vi "mainOCR.vi"() -> ()   [LabVIEW 2025]
uses:
  ocr/ocrParameters.ctl
  ocr/ocr.lvclass
  D:/Test/adslvPackageDev/adstoolkit/tcv/tcv.lvclass
panel:
  out "loadImgSucc":string
  out "succ 2":i32
  in  "Default Parameters":bool
  in  "device":enum16{"CPU", "GPU0"}(ring)
  out "InitRecDec Success":string
  out "SetDevice":string
  in  "ocrParameters":T1={"targetSize"=1088, "expandRatio "=1.12, "padPixels "=10, "binThresh"=0.3, "txt_score_thresh"=0.25, "minArea"=12, "cropMargin"=5, "binSize"=32}
  in  "PathImage":path=path "D:/Test/dllTest/images_2"
  out "Image":T2(plugin-control)
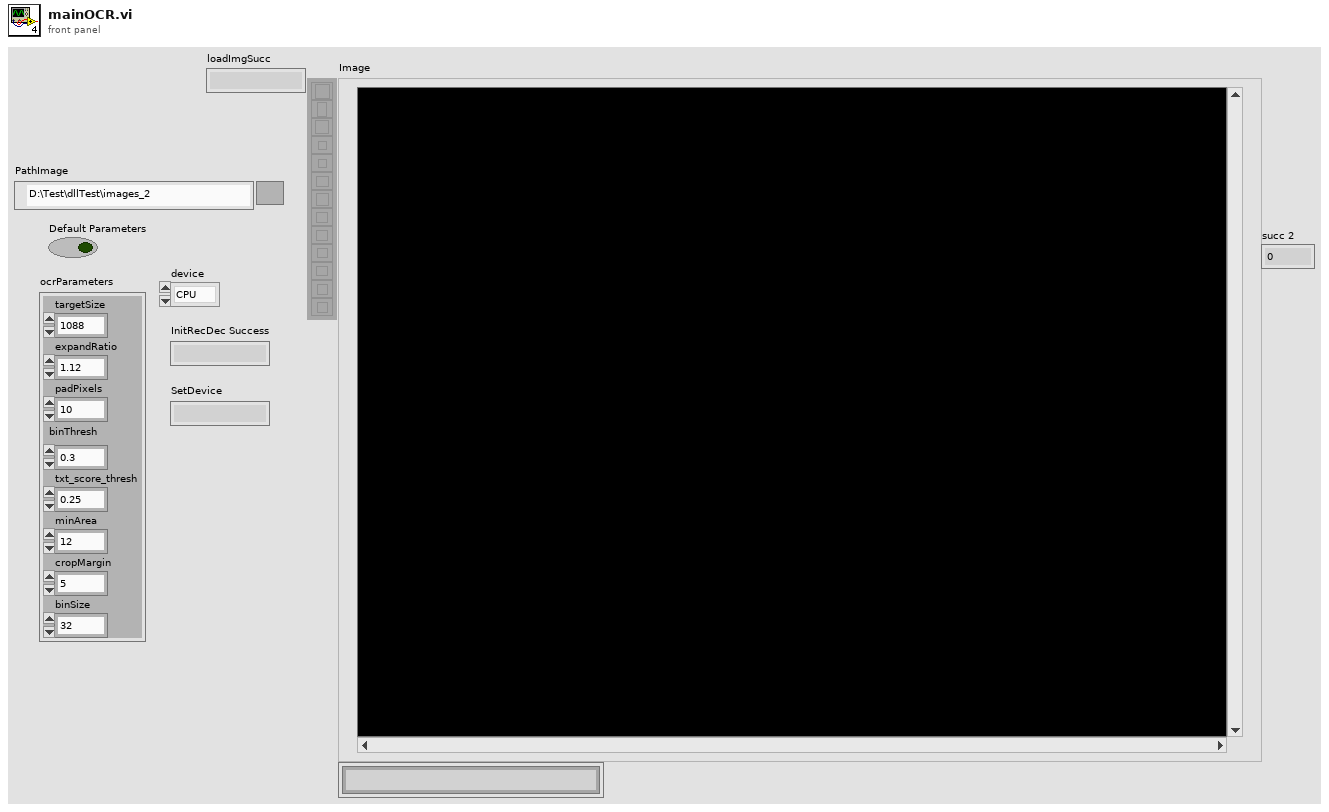
[diagram p1: front panel]
types:
  T1 = typedef "adsOCR.lvlib/ocr.lvclass/ocrParameters.ctl" = cluster{"targetSize":i32, "expandRatio ":sgl, "padPixels ":i32, "binThresh":sgl, "txt_score_thresh":sgl, "minArea":i32, "cropMargin":i32, "binSize":i32}
  T2 = typedef "IMAQ Image.ctl" = refnum<image>
  T3 = typedef "adsOCR.lvlib/ocr.lvclass/TextDecRecResult2L.ctl" = cluster{"imgIdx":i32, "TLx":i32, "TLy":i32, "BRx":i32, "BRy":i32, "angle":sgl, "txtLen":i32}
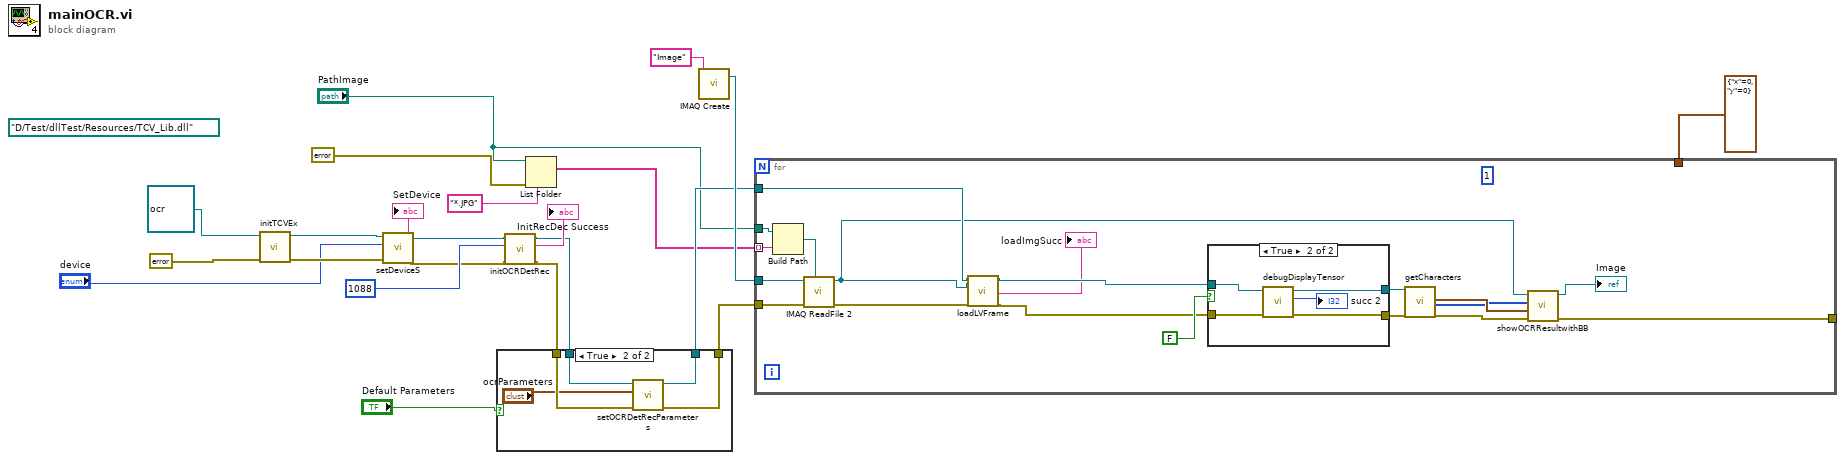
[diagram p0: block diagram]
diagram:
  (unwired) path "D:/Test/dllTest/Resources/TCV_Lib.dll" ("path in")
  n1 = call-dynamic "initTCVEx.vi"("error in (no error)"=errorcluster {"status"=FALSE, "code"=0, "source"=""}, "tcv in"=refnum<class "ocr.lvclass"> refnum ("ocr in")) -> ("error out"=w15:errorcluster, "tcv out"=w16:refnum<class "ocr.lvclass">)  [unwired: 8 in]
  n2 = call-dynamic "setDeviceS.vi"("error in (no error)"=w15, "devices"="device", "tcv in"=w16) -> ("error out"=w4:errorcluster, "SetDevice"=→"SetDevice":string, "tcv out"=w5:refnum<class "ocr.lvclass">)  [unwired: 6 in]
  n3 = call "initOCRDetRec.vi"("error in (no error)"=w4, "targetSize"=1088, "tcv in"=w5) -> ("error out"=w2:errorcluster, "InitRecDec Success"=→"InitRecDec Success":string, "ocr out"=w1:refnum<class "ocr.lvclass">)  [unwired: 5 in, 1 out]
  n4 = case shown="True" "Default Parameters" {
    tunnel: w1 -> [w24 w29]
    tunnel: [w24 w28] -> w14
    tunnel: w2 -> [w23 w27]
    tunnel: [w23 w26] -> w13
    frame False {
    }
    frame True {
      n5 = call-dynamic "setOCRDetRecParameters.vi"("error in (no error)"=w27, "ocrParameters"="ocrParameters", "ocr in"=w29) -> ("error out"=w26:errorcluster, "ocr out"=w28:refnum<class "ocr.lvclass">)  [unwired: 5 in, 2 out]
    }
  }
  n6 = List Folder(path="PathImage", pattern="*.JPG", error in=errorcluster {"status"=FALSE, "code"=0, "source"=""}) -> (filenames=w9:string[])  [unwired: 1 in, 3 out]
  n7 = call "IMAQ Create"("Image Name"="Image") -> ("New Image"=w21:T2)  [unwired: 4 in, 1 out]
  n8 = for {
    tunnel: "PathImage" -> [w48]
    tunnel: w21 -> [w46]
    tunnel: cluster{"x":i32, "y":i32} {"x"=0, "y"=0} -> [_]
    tunnel: w14 -> [w37]
    tunnel: w13 -> [w45]
    tunnel: w9 -> [w44] mode=indexing
    tunnel: [w39] -> _
    (unwired) 1 ("numberofImgs")
    n9 = Build Path(base path=w48, name or relative path=w44) -> (appended path=w47:path)
    n10 = call "IMAQ ReadFile 2"("File Path"=w47, "error in (no error)"=w45, "Image"=w46) -> ("error out"=w35:errorcluster, "Image Out"=w36:T2)  [unwired: 4 in, 3 out]
    n11 = call-dynamic "loadLVFrame.vi"("tcv in"=w37, "Image"=w36, "error in (no error)"=w35) -> ("tcv out"=w34:refnum<class "ocr.lvclass">, "loadImgSucc"=→"loadImgSucc":string, "error out"=w32:errorcluster)  [unwired: 13 in, 1 out]
    n12 = case shown="True" FALSE {
      tunnel: [w50 w55] -> w43
      tunnel: [w49 w54] -> w42
      tunnel: w34 -> [w50 w52]
      tunnel: w32 -> [w49 w51]
      frame False {
      }
      frame True {
        n13 = call-dynamic "debugDisplayTensor.vi"("error in (no error)"=w51, "tcv in"=w52) -> ("error out"=w54:errorcluster, "succ"=→"succ 2":i32, "tcv out"=w55:refnum<class "ocr.lvclass">)  [unwired: 6 in, 1 out]
      }
    }
    n14 = call-dynamic "getCharacters.vi"("ocr in"=w43, "error in (no error)"=w42) -> ("TextDecRecResult2L"=w31:T3[], "chars"=w30:u8[], "error out"=w38:errorcluster)  [unwired: 12 in, 3 out]
    n15 = call "showOCRResultwithBB.vi"("error in"=w38, "Array"=w31, "chars"=w30, "Image in"=w36) -> ("error out"=w39:errorcluster, "Image out"=→"Image":T2)  [unwired: 6 in]
  }
